vi "CIVI Set Frequency Example.vi"() -> ()   [LabVIEW 2026]
panel:
  in  "Frequency Setpoint (Hz)":i32=774000
  out "Operation Complete":string
  out "SCPI Error Response":string
  out "Frequency Response":string
  out "IDN Response":string
  out "error out":errorcluster
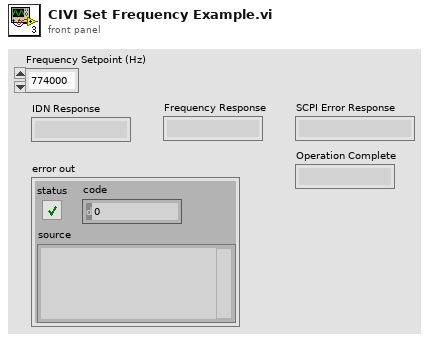
[diagram p1: front panel]
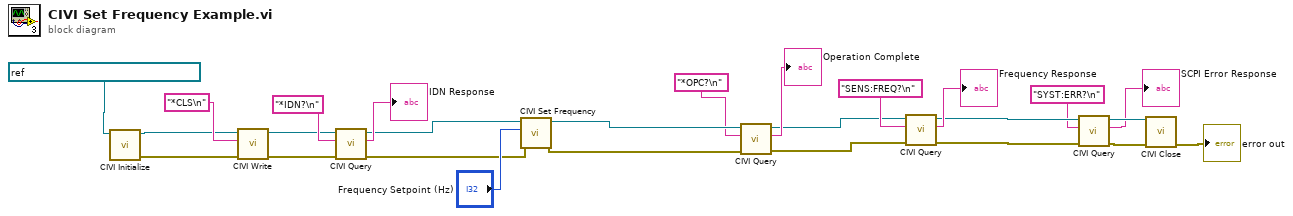
[diagram p0: block diagram]
diagram:
  n1 = call "CIVI Initialize.vi"("VISA Resource Name"=refnum<visa-resource-name> "TCPIP0::127.0.0.1::5025::SOCKET") -> ("error out"=w20:errorcluster, "VISA Session out"=w16:refnum<visa-resource-name>)  [unwired: 9 in]
  n2 = call "CIVI Write.vi"("error in"=w20, "write buffer"="*CLS\n", "VISA Session in"=w16) -> ("error out"=w18:errorcluster, "VISA Session out"=w19:refnum<visa-resource-name>)  [unwired: 7 in]
  n3 = call "CIVI Query.vi"("error in"=w18, "write buffer"="*IDN?\n", "VISA Session in"=w19) -> ("error out"=w1:errorcluster, "read buffer"=→"IDN Response":string, "VISA Session out"=w3:refnum<visa-resource-name>)  [unwired: 6 in]
  n4 = call "CIVI Set Frequency.vi"("error in (no error)"=w1, "Frequency Setpoint (Hz)"="Frequency Setpoint (Hz)", "VISA Refnum in"=w3) -> ("error out"=w8:errorcluster, "VISA Refnum out"=w9:refnum<visa-resource-name>)  [unwired: 7 in]
  n5 = call "CIVI Query.vi"("error in"=w8, "write buffer"="*OPC?\n", "VISA Session in"=w9) -> ("error out"=w4:errorcluster, "read buffer"=→"Operation Complete":string, "VISA Session out"=w5:refnum<visa-resource-name>)  [unwired: 6 in]
  n6 = call "CIVI Query.vi"("error in"=w4, "write buffer"="SENS:FREQ?\n", "VISA Session in"=w5) -> ("error out"=w12:errorcluster, "read buffer"=→"Frequency Response":string, "VISA Session out"=w14:refnum<visa-resource-name>)  [unwired: 6 in]
  n7 = call "CIVI Query.vi"("error in"=w12, "write buffer"="SYST:ERR?\n", "VISA Session in"=w14) -> ("error out"=w13:errorcluster, "read buffer"=→"SCPI Error Response":string, "VISA Session out"=w15:refnum<visa-resource-name>)  [unwired: 6 in]
  n8 = call "CIVI Close.vi"("error in"=w13, "VISA Session in"=w15) -> ("error out"=→"error out":errorcluster)  [unwired: 9 in]
